vi "Configure Band selector Visibility.vi"(8 "error in (no error)":errorcluster, 10 "Number of Bands in":T2=4 min=3 max=6 step=1, 11 "Selec Refn":T1) -> (0 "error out":errorcluster, 2 "Number of Bands out":T2=4 min=3 max=6 step=1)   [LabVIEW 2018, in "Front Panel Interface.lvlib"]
doc: "Configures the visibility of the resistor band selector controls on the Front Panel according to the selected number of bands.\n\nThe VI receives the <b>Number of Bands in</b> and a cluster of <b>Selec Refn</b>. It determines which band selectors must be visible for 3-, 4-, 5-, and 6-band resistor configurations and updates the <b>Visible</b> property of each Enum control. <b>Number of Bands out</b> passes through the value of <b>Number of Bands in</b>.\n\nThe VI only configures Front Panel visibility. It does not modify the value or configuration of any band selector."
uses:
  Front Panel Interface.lvlib
  Number of Bands--numeric.ctl
  Resistor Controls/Selectors Refnums--cluster.ctl
  Resistor Controls/Digit--enum.ctl
  Resistor Controls/Multiplier--enum.ctl
  Resistor Controls/Tolerance--enum.ctl
  Resistor Controls/Temp Coefficient--enum.ctl
  Resistor Controls/Resistance Controls.lvlib
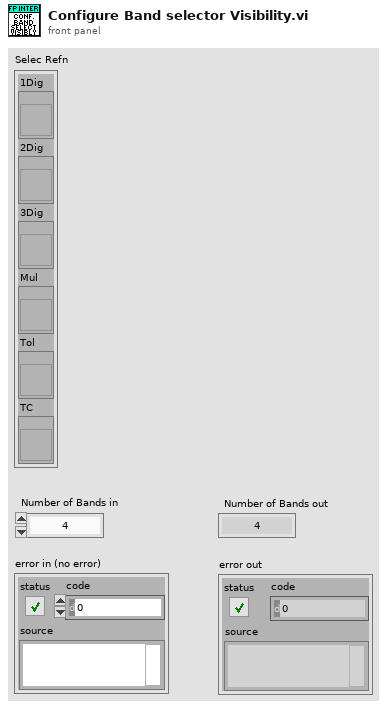
[diagram p1: front panel]
types:
  T1 = typedef "Resistance Controls.lvlib/Selectors Refnums--cluster.ctl" = cluster{"1Dig":refnum<vi>, "2Dig":refnum<vi>, "3Dig":refnum<vi>, "Mul":refnum<vi>, "Tol":refnum<vi>, "TC":refnum<vi>}
  T2 = typedef "Number of Bands--numeric.ctl" = u8
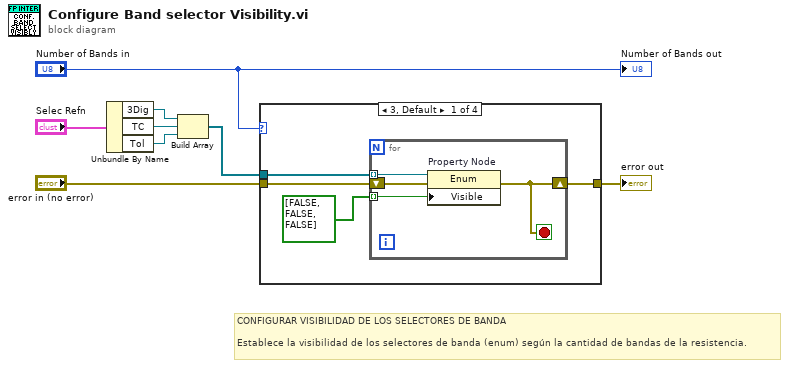
[diagram p0: block diagram]
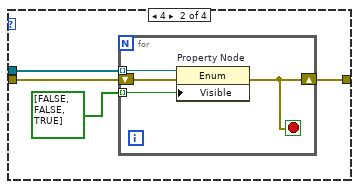
[diagram p2: hidden frame]
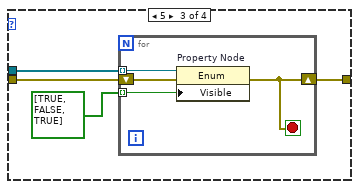
[diagram p3: hidden frame]
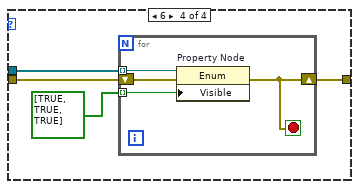
[diagram p4: hidden frame]
diagram:
  # "CONFIGURAR VISIBILIDAD DE LOS SELECTORES DE BANDA\n\nEstablece la visibilidad de los selectores de banda (enum) según la cantidad de bandas de la resistencia."
  n1 = Unbundle By Name("Selec Refn") -> ("3Dig"=w3:refnum<vi>, "TC"=w4:refnum<vi>, "Tol"=w2:refnum<vi>)
  n2 = Build Array(w3, w4, w2) -> (w1:refnum<vi>[])
  n3 = case shown="3, Default" "Number of Bands in" {
    tunnel: [w12 w18 w28 w35] -> w8
    tunnel: "error in (no error)" -> [w11 w19 w27 w36]
    tunnel: w1 -> [w10 w17 w26 w34]
    frame 3, Default {
      n4 = for {
        tunnel: bool[] [FALSE, FALSE, FALSE] -> [w13] mode=indexing
        shift-right: [w15] -> w12
        shift-left: w11 -> [w16]
        tunnel: w10 -> [w14] mode=indexing
        stop <- w15 stop-if-true
        n5 = property on="Property Node" class="Enum"(reference=w14, error in=w16, "Visible"=w13) -> (error out=w15:errorcluster)  [unwired: 1 out]
      }
    }
    frame 4 {
      n6 = for {
        tunnel: bool[] [FALSE, FALSE, TRUE] -> [w21] mode=indexing
        shift-right: [w23] -> w18
        shift-left: w19 -> [w24]
        tunnel: w17 -> [w22] mode=indexing
        stop <- w23 stop-if-true
        n7 = property on="Property Node" class="Enum"(reference=w22, error in=w24, "Visible"=w21) -> (error out=w23:errorcluster)  [unwired: 1 out]
      }
    }
    frame 5 {
      n8 = for {
        tunnel: bool[] [TRUE, FALSE, TRUE] -> [w29] mode=indexing
        shift-right: [w31] -> w28
        shift-left: w27 -> [w32]
        tunnel: w26 -> [w30] mode=indexing
        stop <- w31 stop-if-true
        n9 = property on="Property Node" class="Enum"(reference=w30, error in=w32, "Visible"=w29) -> (error out=w31:errorcluster)  [unwired: 1 out]
      }
    }
    frame 6 {
      n10 = for {
        tunnel: bool[] [TRUE, TRUE, TRUE] -> [w37] mode=indexing
        shift-right: [w39] -> w35
        shift-left: w36 -> [w40]
        tunnel: w34 -> [w38] mode=indexing
        stop <- w39 stop-if-true
        n11 = property on="Property Node" class="Enum"(reference=w38, error in=w40, "Visible"=w37) -> (error out=w39:errorcluster)  [unwired: 1 out]
      }
    }
  }
  "error out" <- w8
  "Number of Bands out" <- "Number of Bands in"
